vi "GetControlValue.vi"(7 "Data":T1, 8 "error in (no error)":errorcluster, 10 "Datatype":string, 11 "Control index":i32) -> (0 "error out":errorcluster, 3 "Offline Value":variant)   [LabVIEW 2017]
uses:
  Ctrl/Data.ctl
  Ctrl/Caps.ctl
  Ctrl/Property.ctl
  Ctrl/PhysicalChannel.ctl
  Ctrl/Register.ctl
  Ctrl/Bitfield.ctl
  Ctrl/Scale.ctl
  Ctrl/ScaleType.ctl
  Ctrl/Enum.ctl
  Ctrl/EnumValue.ctl
  API/Parser/Paser.lvlib
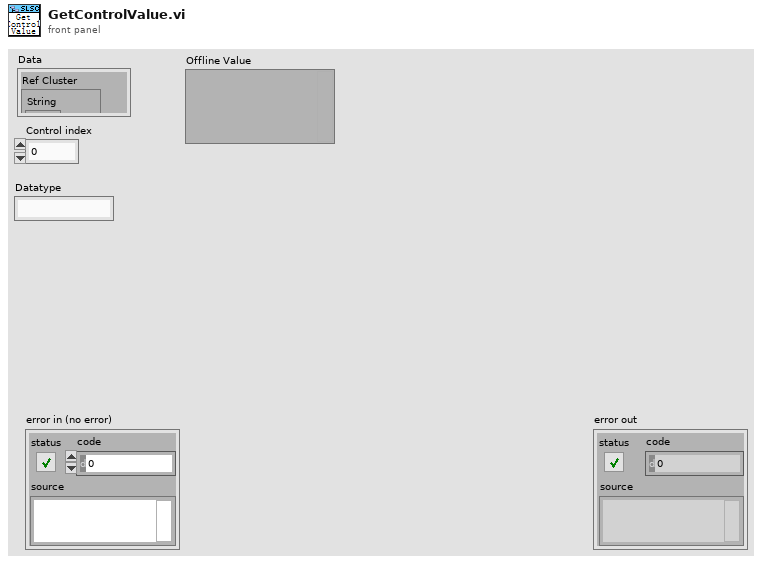
[diagram p1: front panel]
types:
  T1 = typedef "Data.ctl" = cluster{"Ref Cluster":cluster{"String":refnum<vi>, "U8":refnum<vi>, "I8":refnum<vi>, "U32":refnum<vi>, "I32":refnum<vi>, "U64":refnum<vi>, "I64":refnum<vi>, "Ring":refnum<vi>, "DBL":refnum<vi>, "Add":refnum<vi>, "Remove":refnum<vi>, "Property tree":refnum<vi>, "confirm":refnum<vi>}, "JSON Text":string, "Original JSON Text":string, "Caps":T2, "SLSC Output Tree":cluster{"Left Cell String":string, "Child Text":string[], "Child Tag":string, "Item Indent":i32, "Child Only?":bool, "Glyph Index":i32, "offline value":variant}[], "Ref Index and Control Type":cluster{"index":i32, "Datatype":string}, "Selected Type and name":cluster{"Selected Type":enum16{"Property", "Physical Channel", "Other"}, "Selected Property Name":string}, "Update whole Tree?":bool}
  T2 = typedef "Caps.ctl" = cluster{"properties":T3[], "physical channels":T4[], "registers":T5[], "scales":T7[], "enums":T9[], "productName":string}
  T3 = typedef "Property.ctl" = cluster{"name":string, "bitfield":string, "value":variant, "dataType":string, "min":variant, "max":variant, "scale":string, "access":string}
  T4 = typedef "PhysicalChannel.ctl" = cluster{"name":string, "properties":T3[]}
  T5 = typedef "Register.ctl" = cluster{"name":string, "address":i32, "size":i32, "bitfields":T6[], "initialValue":variant, "connectedProperties":string[]}
  T6 = typedef "Bitfield.ctl" = cluster{"name":string, "offset":i32, "size":i32, "signed":bool}
  T7 = typedef "Scale.ctl" = cluster{"name":string, "type":T8, "params":variant}
  T8 = typedef "ScaleType.ctl" = enum16{"NoScale", "Table", "Polynomial", "Linear"}
  T9 = typedef "Enum.ctl" = cluster{"name":string, "values":T10[]}
  T10 = typedef "EnumValue.ctl" = cluster{"name":string, "value":i32}
  T11 = cluster{"Left Cell String":string, "Child Text":string[], "Child Tag":string, "Item Indent":i32, "Child Only?":bool, "Glyph Index":i32, "offline value":variant}[]
  T12 = cluster{"String":refnum<vi>, "U8":refnum<vi>, "I8":refnum<vi>, "U32":refnum<vi>, "I32":refnum<vi>, "U64":refnum<vi>, "I64":refnum<vi>, "Ring":refnum<vi>, "DBL":refnum<vi>, "Add":refnum<vi>, "Remove":refnum<vi>, "Property tree":refnum<vi>, "confirm":refnum<vi>}
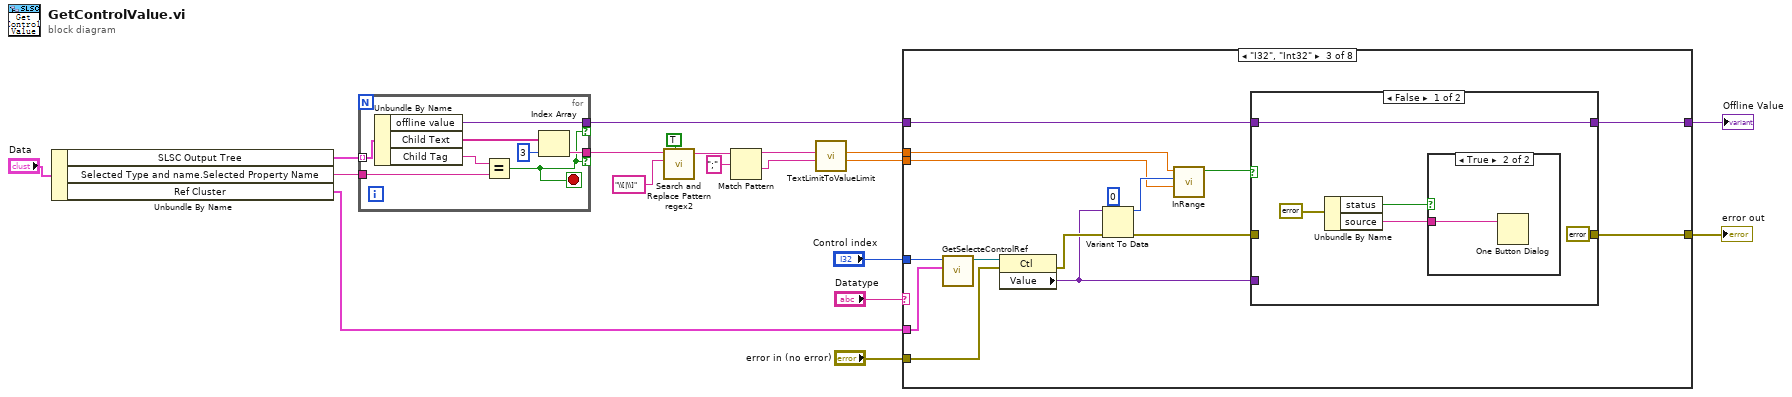
[diagram p0: block diagram]
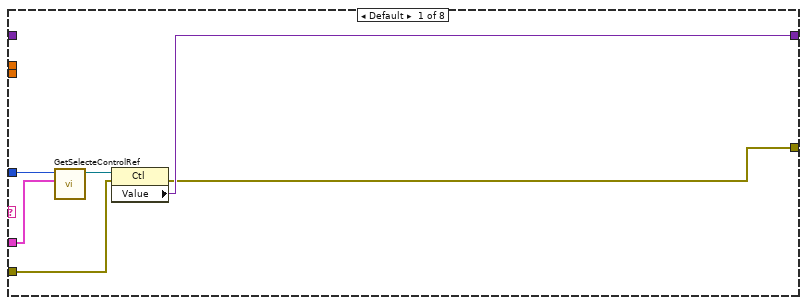
[diagram p2: hidden frame]
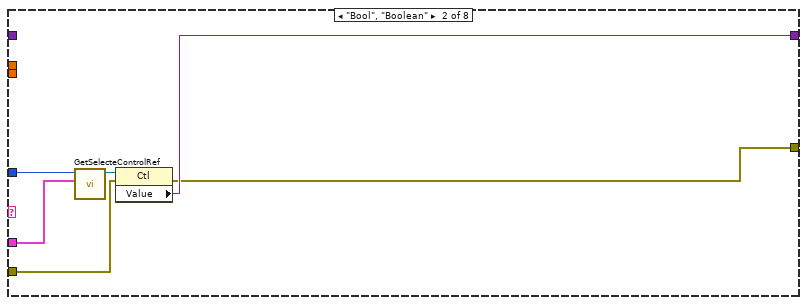
[diagram p3: hidden frame]
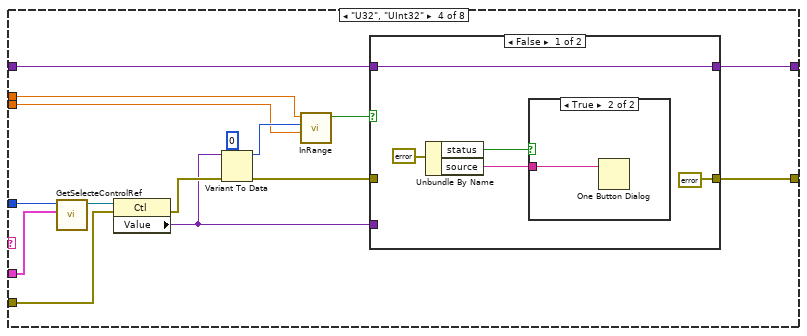
[diagram p6: hidden frame]
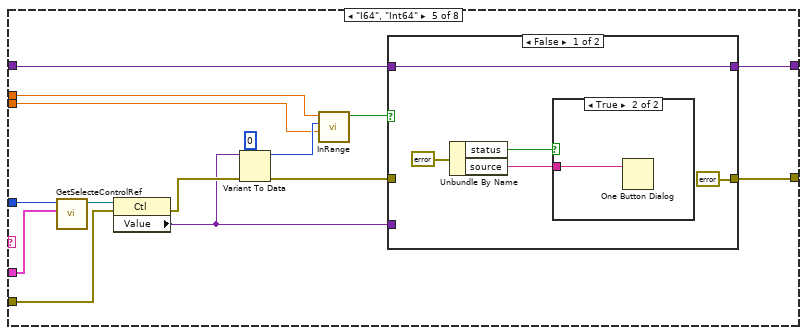
[diagram p9: hidden frame]
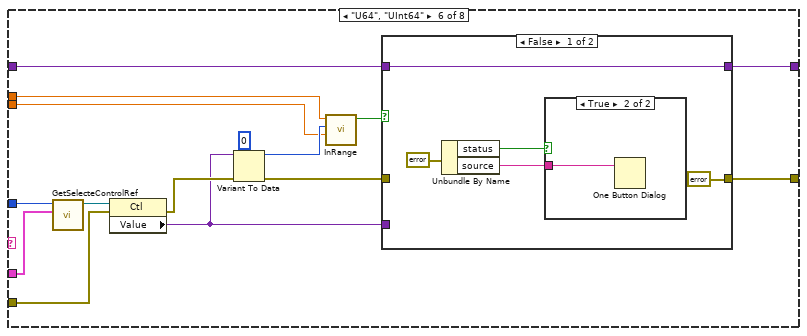
[diagram p12: hidden frame]
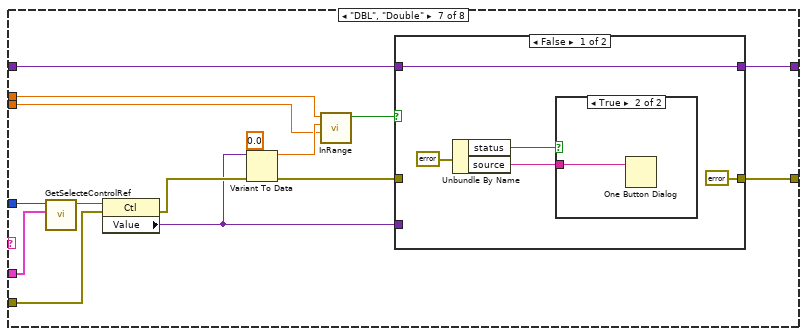
[diagram p15: hidden frame]
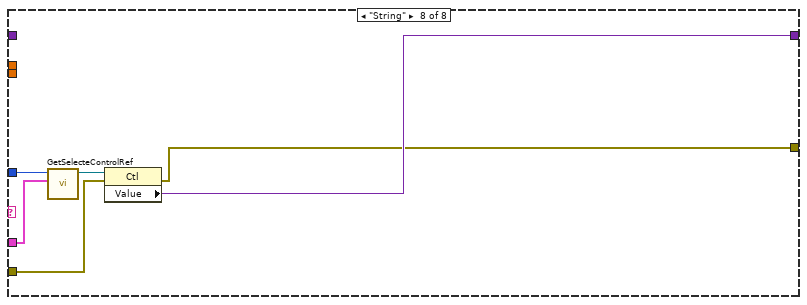
[diagram p18: hidden frame]
diagram:
  n1 = Unbundle By Name("Data") -> ("SLSC Output Tree"=w15:T11, "Selected Type and name.Selected Property Name"=w14:string, "Ref Cluster"=w1:T12)
  n2 = for {
    tunnel: w15 -> [w27] mode=indexing
    tunnel: w14 -> [w26]
    tunnel: [w23] -> w11 if=w20
    tunnel: [w21] -> w4 if=w20
    stop <- w20 stop-if-true
    n3 = Unbundle By Name(w27) -> ("offline value"=w21:variant, "Child Text"=w25:string[], "Child Tag"=w22:string)
    n4 = Equal?(x=w22, y=w26) -> (x = y?=w20:bool)
    n5 = Index Array(array=w25, index=3) -> (element=w23:string)
  }
  n6 = call "Search and Replace Pattern regex2.vi"("replace all? (F)"=TRUE, "regular expression (\"\")"="\\[|\\]" ("regular expression (\"\")"), "string"=w11) -> ("result string"=w10:string)  [unwired: 6 in, 2 out]
  n7 = Match Pattern(string=w10, regular expression=";") -> (before substring=w8:string, after substring=w7:string)  [unwired: 1 in, 2 out]
  n8 = call "TextLimitToValueLimit.vi"("max"=w7, "min"=w8) -> ("max"=w5:dbl, "min"=w6:dbl)  [unwired: 8 in]
  n9 = case shown="\"I32\", \"Int32\"" "Datatype" {
    tunnel: "Control index" -> [w33 w38 w53 w77 w100 w123 w146 w160]
    tunnel: w1 -> [w28 w37 w52 w76 w99 w122 w145 w159]
    tunnel: "error in (no error)" -> [w31 w36 w51 w74 w97 w120 w143 w157]
    tunnel: w6 -> [_ _ w41 w63 w87 w110 w133 _]
    tunnel: w5 -> [_ _ w40 w64 w86 w109 w132 _]
    tunnel: w4 -> [_ _ w48 w71 w94 w117 w140 _]
    tunnel: [w30 w35 w47 w70 w91 w114 w139 w156] -> w3
    tunnel: [w29 w34 w44 w69 w90 w113 w138 w155] -> w2
    frame Default {
      n10 = call "GetSelecteControlRef.vi"("Ref Cluster"=w28, "index"=w33) -> ("Control out"=w32:refnum<vi>)  [unwired: 9 in]
      n11 = property class="Ctl"(reference=w32, error in=w31) -> (error out=w29:errorcluster, "Value"=w30:variant)  [unwired: 1 out]
    }
    frame "Bool", "Boolean" {
      n12 = call "GetSelecteControlRef.vi"("Ref Cluster"=w37, "index"=w38) -> ("Control out"=w39:refnum<vi>)  [unwired: 9 in]
      n13 = property class="Ctl"(reference=w39, error in=w36) -> (error out=w34:errorcluster, "Value"=w35:variant)  [unwired: 1 out]
    }
    frame "I32", "Int32" {
      n14 = call "GetSelecteControlRef.vi"("Ref Cluster"=w52, "index"=w53) -> ("Control out"=w54:refnum<vi>)  [unwired: 9 in]
      n15 = property class="Ctl"(reference=w54, error in=w51) -> (error out=w49:errorcluster, "Value"=w46:variant)  [unwired: 1 out]
      n16 = Variant To Data(error in=w49, type=0, Variant=w46) -> (data=w42:i32, error out=w45:errorcluster)
      n17 = call "InRange.vi"("Max"=w40, "Value"=w42, "Min"=w41) -> ("Boolean"=w43:bool)  [unwired: 8 in]
      n18 = case shown="False" w43 {
        tunnel: w48 -> [w59 _]
        tunnel: [w59 w62] -> w47
        tunnel: w46 -> [_ w62]
        tunnel: [errorcluster {"status"=FALSE, "code"=0, "source"=""} ("error out") w61] -> w44
        tunnel: w45 -> [_ w61]
        frame False {
          n19 = Unbundle By Name(errorcluster {"status"=TRUE, "code"=-995, "source"="Input value out of range"} ("error out")) -> ("status"=w58:bool, "source"=w57:string)
          n20 = case shown="True" w58 {
            tunnel: w57 -> [_ w60]
            frame False {
            }
            frame True {
              n21 = One Button Dialog(message=w60) -> ()  [unwired: 1 in, 1 out]
            }
          }
        }
        frame True {
        }
      }
    }
    frame "U32", "UInt32" {
      n22 = call "GetSelecteControlRef.vi"("Ref Cluster"=w76, "index"=w77) -> ("Control out"=w75:refnum<vi>)  [unwired: 9 in]
      n23 = property class="Ctl"(reference=w75, error in=w74) -> (error out=w68:errorcluster, "Value"=w67:variant)  [unwired: 1 out]
      n24 = Variant To Data(error in=w68, type=0, Variant=w67) -> (data=w65:i32, error out=w72:errorcluster)
      n25 = call "InRange.vi"("Max"=w64, "Value"=w65, "Min"=w63) -> ("Boolean"=w66:bool)  [unwired: 8 in]
      n26 = case shown="False" w66 {
        tunnel: w71 -> [w82 _]
        tunnel: [w82 w85] -> w70
        tunnel: w67 -> [_ w85]
        tunnel: [errorcluster {"status"=FALSE, "code"=0, "source"=""} ("error out") w84] -> w69
        tunnel: w72 -> [_ w84]
        frame False {
          n27 = Unbundle By Name(errorcluster {"status"=TRUE, "code"=-995, "source"="Input value out of range"} ("error out")) -> ("status"=w81:bool, "source"=w80:string)
          n28 = case shown="True" w81 {
            tunnel: w80 -> [_ w83]
            frame False {
            }
            frame True {
              n29 = One Button Dialog(message=w83) -> ()  [unwired: 1 in, 1 out]
            }
          }
        }
        frame True {
        }
      }
    }
    frame "I64", "Int64" {
      n30 = call "GetSelecteControlRef.vi"("Ref Cluster"=w99, "index"=w100) -> ("Control out"=w98:refnum<vi>)  [unwired: 9 in]
      n31 = property class="Ctl"(reference=w98, error in=w97) -> (error out=w93:errorcluster, "Value"=w92:variant)  [unwired: 1 out]
      n32 = Variant To Data(error in=w93, type=0, Variant=w92) -> (data=w88:i32, error out=w95:errorcluster)
      n33 = call "InRange.vi"("Max"=w86, "Value"=w88, "Min"=w87) -> ("Boolean"=w89:bool)  [unwired: 8 in]
      n34 = case shown="False" w89 {
        tunnel: w94 -> [w105 _]
        tunnel: [w105 w108] -> w91
        tunnel: w92 -> [_ w108]
        tunnel: [errorcluster {"status"=FALSE, "code"=0, "source"=""} ("error out") w107] -> w90
        tunnel: w95 -> [_ w107]
        frame False {
          n35 = Unbundle By Name(errorcluster {"status"=TRUE, "code"=-995, "source"="Input value out of range"} ("error out")) -> ("status"=w104:bool, "source"=w103:string)
          n36 = case shown="True" w104 {
            tunnel: w103 -> [_ w106]
            frame False {
            }
            frame True {
              n37 = One Button Dialog(message=w106) -> ()  [unwired: 1 in, 1 out]
            }
          }
        }
        frame True {
        }
      }
    }
    frame "U64", "UInt64" {
      n38 = call "GetSelecteControlRef.vi"("Ref Cluster"=w122, "index"=w123) -> ("Control out"=w121:refnum<vi>)  [unwired: 9 in]
      n39 = property class="Ctl"(reference=w121, error in=w120) -> (error out=w116:errorcluster, "Value"=w115:variant)  [unwired: 1 out]
      n40 = Variant To Data(error in=w116, type=0, Variant=w115) -> (data=w111:i32, error out=w118:errorcluster)
      n41 = call "InRange.vi"("Max"=w109, "Value"=w111, "Min"=w110) -> ("Boolean"=w112:bool)  [unwired: 8 in]
      n42 = case shown="False" w112 {
        tunnel: w117 -> [w128 _]
        tunnel: [w128 w131] -> w114
        tunnel: w115 -> [_ w131]
        tunnel: [errorcluster {"status"=FALSE, "code"=0, "source"=""} ("error out") w130] -> w113
        tunnel: w118 -> [_ w130]
        frame False {
          n43 = Unbundle By Name(errorcluster {"status"=TRUE, "code"=-995, "source"="Input value out of range"} ("error out")) -> ("status"=w127:bool, "source"=w126:string)
          n44 = case shown="True" w127 {
            tunnel: w126 -> [_ w129]
            frame False {
            }
            frame True {
              n45 = One Button Dialog(message=w129) -> ()  [unwired: 1 in, 1 out]
            }
          }
        }
        frame True {
        }
      }
    }
    frame "DBL", "Double" {
      n46 = call "GetSelecteControlRef.vi"("Ref Cluster"=w145, "index"=w146) -> ("Control out"=w144:refnum<vi>)  [unwired: 9 in]
      n47 = property class="Ctl"(reference=w144, error in=w143) -> (error out=w137:errorcluster, "Value"=w136:variant)  [unwired: 1 out]
      n48 = Variant To Data(error in=w137, type=0.0, Variant=w136) -> (data=w134:dbl, error out=w141:errorcluster)
      n49 = call "InRange.vi"("Max"=w132, "Value"=w134, "Min"=w133) -> ("Boolean"=w135:bool)  [unwired: 8 in]
      n50 = case shown="False" w135 {
        tunnel: w140 -> [w151 _]
        tunnel: [w151 w154] -> w139
        tunnel: w136 -> [_ w154]
        tunnel: [errorcluster {"status"=FALSE, "code"=0, "source"=""} ("error out") w153] -> w138
        tunnel: w141 -> [_ w153]
        frame False {
          n51 = Unbundle By Name(errorcluster {"status"=TRUE, "code"=-995, "source"="Input value out of range"} ("error out")) -> ("status"=w150:bool, "source"=w149:string)
          n52 = case shown="True" w150 {
            tunnel: w149 -> [_ w152]
            frame False {
            }
            frame True {
              n53 = One Button Dialog(message=w152) -> ()  [unwired: 1 in, 1 out]
            }
          }
        }
        frame True {
        }
      }
    }
    frame "String" {
      n54 = call "GetSelecteControlRef.vi"("Ref Cluster"=w159, "index"=w160) -> ("Control out"=w158:refnum<vi>)  [unwired: 9 in]
      n55 = property class="Ctl"(reference=w158, error in=w157) -> (error out=w155:errorcluster, "Value"=w156:variant)  [unwired: 1 out]
    }
  }
  "Offline Value" <- w3
  "error out" <- w2
